vi "Burst Clock (FPGA).vi"() -> ()   [LabVIEW 2021]
uses:
  <vilib>/Platform/TimedLoop/XDataNode/timing_clust.ctl
  <vilib>/Platform/TimedLoop/XDataNode/nitl_modes.ctl
  <vilib>/Platform/TimedLoop/XDataNode/wakeup.ctl
  States Typedef.ctl
  <vilib>/rvi/Emulation/niFpgaGetClockAttributes.vi
  <vilib>/rvi/Emulation/niFpgaSctlEmulationGetInTimedLoop.vi
  <vilib>/rvi/Emulation/niFpgaEmulationReportErrorSimple.vi
  <vilib>/rvi/eio/common/nirviEmuTemplateMethod_errors.vi
  <vilib>/rvi/Emulation/niFpgaCriticalErrorInLSC.vi
  <vilib>/rvi/interface/RandomDataEmulation/niFpgaRandomDataHandleErrors.vi
  <vilib>/rvi/DataTransferAndStorage/Container/Common/niFpgaContainerExecOnDevCompGetState.vi
  <vilib>/rvi/Emulation/niFpgaEmulationIsFPGAContextNoSignature.vi
  <vilib>/rvi/errors/niFpgaSetErrorForExecOnDevCompSimple.vi
  <vilib>/rvi/eio/common/nirviEmuReportErrorAndStop.vi
  <vilib>/rvi/DataTransferAndStorage/Container/Common/niFpgaContainerGetUniqueNameForEmu.vi
  <vilib>/rvi/FIFO/Fifo_Resource/nirvififoEmulationSetSize.vi
  <vilib>/rvi/FIFO/Fifo_Resource/nirviFifoEmulationQueueMgr.vi
  <instcachedir>/0/nirviFifoEmulationQueueMgr_E5CAEC123FF24DC58D834DCA3CDAA9B5.lvgen/nirviFifoEmulationQueueMgr_E5CAEC123FF24DC58D834DCA3CDAA9B5_006.vi
  <vilib>/rvi/FIFO/Fifo_Resource/nirvififoEmulationDetermineInputValidOut.vi
  <vilib>/rvi/FIFO/Fifo_Resource/nirvififoEmulationCreateLock.vi
  <vilib>/rvi/Emulation/niFpgaProcessEmulError.vi
  <vilib>/rvi/FIFO/Fifo_Resource/nirvififoEmulationObtainLock.vi
  <vilib>/rvi/FIFO/Fifo_Resource/nirvififoEmulationReleaseLock.vi
  <vilib>/rvi/occurrence/nirviWaitOnOccurrenceBase.vi
  <vilib>/rvi/errors/nirviReportUnexpectedCaseInternalError.vi
  <vilib>/rvi/errors/nirviReportUnexpectedCaseInternalError (U32).vi
  <vilib>/Utility/error.llb/Clear Errors.vi
  <vilib>/eio/EIONode/EIONode.xnode
  <vilib>/Platform/TimedLoop/XDataNode/XDataNode.xnode
  <vilib>/rvi/DataTransferAndStorage/Container/XNode/niFpgaContainer.xnode
  <vilib>/rvi/interface/RandomDataEmulation/nirviRandomDataFpgaReadWriteTemplate.vi
  <vilib>/rvi/FIFO/Fifo_Resource/niFpgaFifoEmulationRefIn.vi
  <vilib>/Platform/TimedLoop/XDataNode/XDNodeRunTimeDep.lvlib
  <instrlib>/_niInstr/Basic Elements/v1/FPGA/niInstr Basic Elements v1 FPGA.lvlib
panel:
  out "Set Voltage Done":bool
  out "IO Enabled":bool
  in  "Go":bool
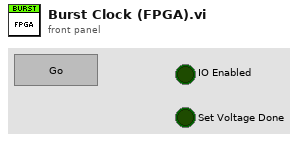
[diagram p1: front panel]
types:
  T1 = cluster{"Outputting Count":u16, "Not Outputting Count":u16, "Outputting Max":u16, "Not Outputting Max":u16, "Num of Bursts Count":u32, "Num of Bursts Max":u32}
  T2 = typedef "States Typedef.ctl" = enum16{"Idle (0)", "Read FIFO (1)", "Outputting (2)", "Not Outputting (3)"}
  T3 = typedef "XDNodeRunTimeDep.lvlib/timing_clust.ctl" = cluster{"Expected End [f-1]":u64, "Actual End [f-1]":u64, "Finished Late? [f-1]":bool, "Expected End [i-1]":u64, "Actual End [i-1]":u64, "Finished Late? [i-1]":bool, "Expected Start [i]":u64, "Actual Start [i]":u64, "Expected Start [f]":u64, "Actual Start [f]":u64, "Source Name":string, "Structure Name":string, "Period":i64, "Deadline":i64, "Offset":i64, "Start":i64, "Priority":i32, "Timeout":i32, "Mode":T4, "Wakeup Reason":T5, "Error":errorcluster, "Source Type":string, "Secondary Source Type":string, "Global End Time":u64, "Global Start Time":u64, "Frame Duration":u64, "Iteration Duration":u64, "Assigned CPU":i32, "I/O Scan Engine Mode":u32}
  T4 = typedef "XDNodeRunTimeDep.lvlib/nitl_modes.ctl" = enum32{"No Change", "Process missed periods, maintain original phase", "Discard missed periods, maintain original phase", "Process missed periods, ignore original phase", "Discard missed periods, ignore original phase"}
  T5 = typedef "XDNodeRunTimeDep.lvlib/wakeup.ctl" = enum32{"Normal", "Aborted", "Asynchronous wakeup", "Timing source error", "Timed loop error", "Timeout"}
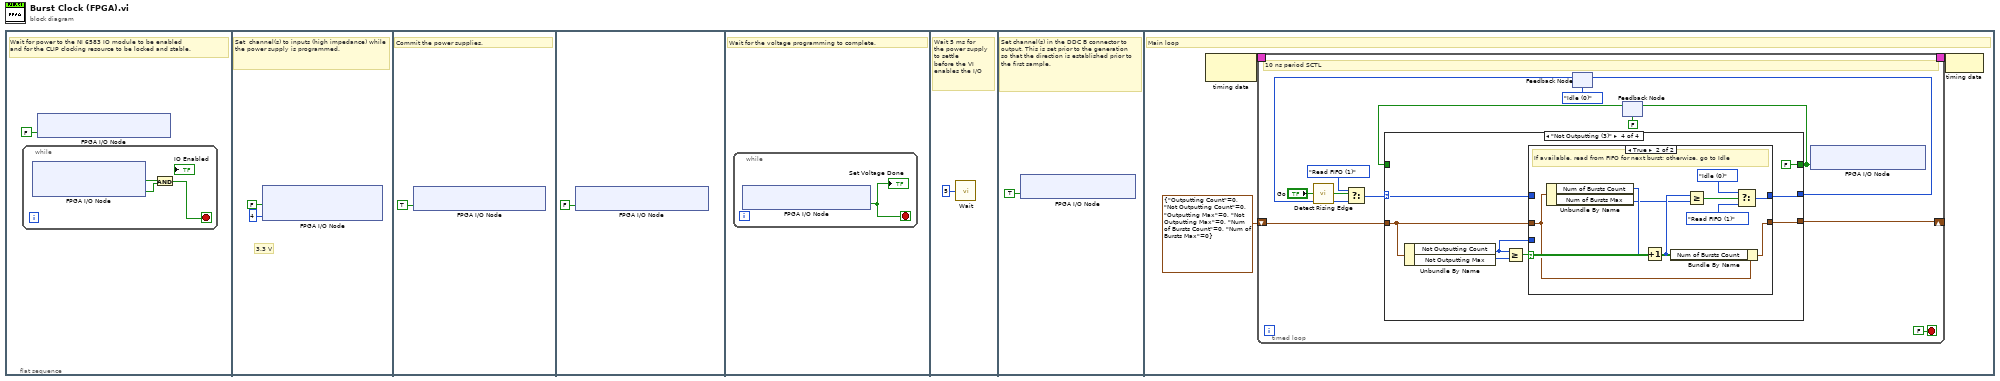
[diagram p0: block diagram]
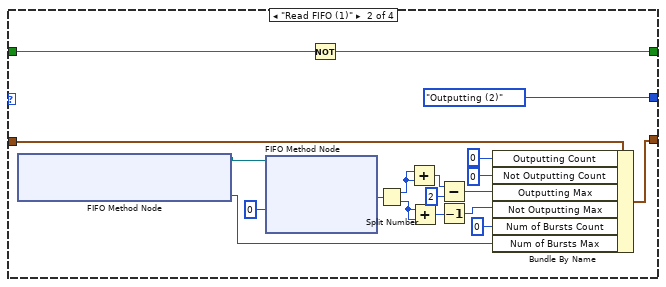
[diagram p3: hidden frame]
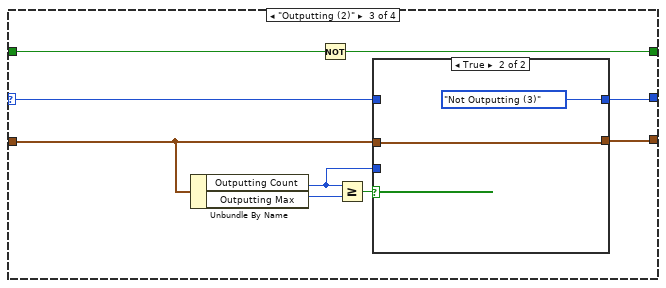
[diagram p4: hidden frame]
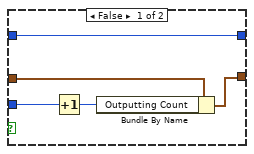
[diagram p5: hidden frame]
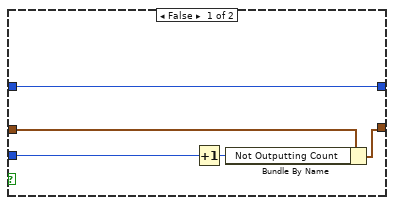
[diagram p6: hidden frame]
diagram:
  n1 = flat-sequence {
    frame #0 {
      # "Wait for power to the NI 6583 IO module to be enabled \nand for the CLIP clocking resource to be locked and stable."
      n2 = while {
        stop <- w2 stop-if-true
        n3 = xnode "FPGA I/O Node"() -> ("IO Module IO Enabled"=w4:bool, "IO Module\\DCM_Locked"=w3:bool)  [unwired: 2 in, 2 out]
        n4 = And(x=w4, y=w3) -> (x .and. y?=w2:bool)
      }
      n5 = xnode "FPGA I/O Node"("IO Module\\Set_Voltage_Family"=FALSE ("IO Module\\Set_Voltage_Family")) -> ()  [unwired: 1 in, 1 out]
    }
    frame #1 {
      # "3.3 V"
      # "Set  channel(s) to inputs (high impedance) while the power supply is programmed."
      n6 = xnode "FPGA I/O Node"("IO Module\\LVDS_Ch0_Dir"=FALSE ("IO Module\\LVDS_Ch0_Dir"), "IO Module\\Voltage_Family"=u8 4 ("IO Module\\Voltage_Family")) -> ()  [unwired: 2 in, 2 out]
    }
    frame #2 {
      # "Commit the power supplies."
      n7 = xnode "FPGA I/O Node"("IO Module\\Set_Voltage_Family"=TRUE ("IO Module\\Set_Voltage_Family")) -> ()  [unwired: 1 in, 1 out]
    }
    frame #3 {
      n8 = xnode "FPGA I/O Node"("IO Module\\Set_Voltage_Family"=FALSE ("IO Module\\Set_Voltage_Family")) -> ()  [unwired: 1 in, 1 out]
    }
    frame #4 {
      # "Wait for the voltage programming to complete."
      n9 = while {
        stop <- w9 stop-if-true
        n10 = xnode "FPGA I/O Node"() -> ("IO Module\\Set_Voltage_Done"=w9:bool)  [unwired: 1 in, 1 out]
        "Set Voltage Done" <- w9
      }
    }
    frame #5 {
      # "Wait 5 ms for \nthe power supply to settle\nbefore the VI enables the I/O"
      n11 = call "Wait"("Count(mSec)"=u16 5) -> ()  [unwired: 1 out]
    }
    frame #6 {
      # "Set channel(s) in the DDC B connector to output. This is set prior to the generation so that the direction is established prior to the first sample."
      n12 = xnode "FPGA I/O Node"("IO Module\\LVDS_Ch0_Dir"=TRUE ("IO Module\\LVDS_Ch0_Dir")) -> ()  [unwired: 1 in, 1 out]
    }
    frame #7 {
      # "Main loop"
      n13 = node-c288() -> (w14:T3)  [unwired: 1 in]
      n14 = timed-loop {
        timing: w14 -> [_]
        timing-out: [_] -> w13
        shift-right: [w26] -> _
        shift-left: T1 {"Outputting Count"=0, "Not Outputting Count"=0, "Outputting Max"=0, "Not Outputting Max"=0, "Num of Bursts Count"=0, "Num of Bursts Max"=0} -> [w27]
        stop <- FALSE stop-if-true
        # "10 ns period SCTL"
        n15 = call <instrlib>:"Detect Rising Edge.vi"("signal"="Go") -> ("edge detected"=w23:bool)  [unwired: 14 in]
        n16 = feedback #1(States_Typedef."Idle (0)" ("Enum")) -> (w18:T2)
        n17 = Select(t=States_Typedef."Read FIFO (1)" ("Enum"), s=w23, f=w18) -> (s? t:f=w16:T2)
        n18 = feedback #2(FALSE) -> (w21:bool)
        n19 = case shown="\"Not Outputting (3)\"" w16 {
          selector: w16 -> [w29 _ w55 w72]
          tunnel: w21 -> [w30 w49 w58 _]
          tunnel: [w30 w33 w57 FALSE] -> w15
          tunnel: [w29 States_Typedef."Outputting (2)" ("Enum") w54 w71] -> w19
          tunnel: w27 -> [w28 w45 w52 w69]
          tunnel: [w28 w42 w53 w70] -> w26
          frame "Idle (0)", Default {
          }
          frame "Read FIFO (1)" {
            n20 = xnode ("FIFO Method Node")() -> ("Number of Elements to Read"=w40:u32, "FIFO Out"=w41:refnum<k21>)  [unwired: 1 in]
            n21 = xnode ("FIFO Method Node")("Timeout"=0, "FIFO In"=w41) -> ("Element"=w46:u32)  [unwired: 2 out]
            n22 = Not(x=w49) -> (.not. x?=w33:bool)
            n23 = Split Number(x=w46) -> (hi(x)=w38:u16, lo(x)=w37:u16)
            n24 = Add(x=w38, y=w38) -> (x+y=w36:u16)
            n25 = Add(x=w37, y=w37) -> (x+y=w32:u16)
            n26 = Subtract(x=w36, y=u16 2) -> (x-y=w34:u16)
            n27 = Decrement(x=w32) -> (x-1=w31:u16)
            n28 = Bundle By Name(cluster=w45, "Outputting Count"=u16 0, "Not Outputting Count"=u16 0, "Outputting Max"=w34, "Not Outputting Max"=w31, "Num of Bursts Count"=u32 0, "Num of Bursts Max"=w40) -> (w42:T1)
          }
          frame "Outputting (2)" {
            n29 = Unbundle By Name(w52) -> ("Outputting Count"=w50:u16, "Outputting Max"=w51:u16)
            n30 = Not(x=w58) -> (.not. x?=w57:bool)
            n31 = Greater Or Equal?(x=w50, y=w51) -> (x >= y?=w56:bool)
            n32 = case shown="True" w56 {
              tunnel: w55 -> [w63 _]
              tunnel: [w63 States_Typedef."Not Outputting (3)" ("Enum")] -> w54
              tunnel: [w59 w64] -> w53
              tunnel: w52 -> [w61 w64]
              tunnel: w50 -> [w62 _]
              frame False {
                n33 = Increment(x=w62) -> (x+1=w60:u16)
                n34 = Bundle By Name(cluster=w61, "Outputting Count"=w60) -> (w59:T1)
              }
              frame True {
              }
            }
          }
          frame "Not Outputting (3)" {
            n35 = Unbundle By Name(w69) -> ("Not Outputting Count"=w67:u16, "Not Outputting Max"=w68:u16)
            n36 = Greater Or Equal?(x=w67, y=w68) -> (x >= y?=w73:bool)
            n37 = case shown="True" w73 {
              tunnel: w72 -> [w78 _]
              tunnel: [w78 w85] -> w71
              tunnel: [w74 w82] -> w70
              tunnel: w69 -> [w76 w83]
              tunnel: w67 -> [w77 _]
              frame False {
                n38 = Increment(x=w77) -> (x+1=w75:u16)
                n39 = Bundle By Name(cluster=w76, "Not Outputting Count"=w75) -> (w74:T1)
              }
              frame True {
                # "If available, read from FIFO for next burst; otherwise, go to Idle"
                n40 = Unbundle By Name(w83) -> ("Num of Bursts Count"=w81:u32, "Num of Bursts Max"=w79:u32)
                n41 = Increment(x=w81) -> (x+1=w80:u32)
                n42 = Bundle By Name(cluster=w83, "Num of Bursts Count"=w80) -> (w82:T1)
                n43 = Greater Or Equal?(x=w80, y=w79) -> (x >= y?=w87:bool)
                n44 = Select(t=States_Typedef."Idle (0)" ("Enum"), s=w87, f=States_Typedef."Read FIFO (1)" ("Enum")) -> (s? t:f=w85:T2)
              }
            }
          }
        }
        n45 = feedback-in #1(w19) -> ()
        n46 = feedback-in #2(w15) -> ()
        n47 = xnode "FPGA I/O Node"("IO Module\\LVDS_Ch0_Wr"=w15) -> ()  [unwired: 1 in, 1 out]
      }
      n48 = node-c288(w13) -> ()
    }
  }
